vi "Get File Path.vi"(8 "error in (no error)":errorcluster caption="错误输入（无错误）", 10 "nRunMode":i32, 11 "nDevId":i32) -> (0 "error out":errorcluster caption="错误输出", 3 "function return":string)   [LabVIEW 2017, in "smncsftmt.lvlib"]
doc: "__declspec(dllexport) char* GetFilePath(int nDevId, int nRunMode);"
uses:
  smncsftmt.lvlib
  smncsftmt.dll
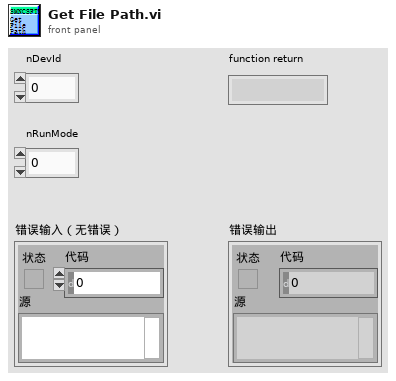
[diagram p1: front panel]
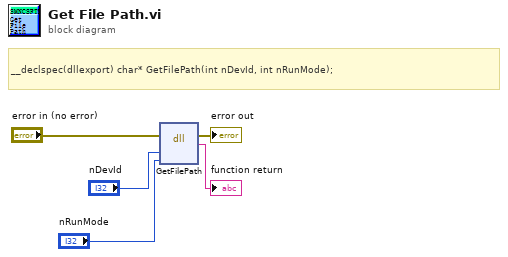
[diagram p0: block diagram]
diagram:
  # "__declspec(dllexport) char* GetFilePath(int nDevId, int nRunMode);"
  n1 = dll-call lib="PTH2oabs CUsersaDesktop\nLABVIEW范例National InstrumentsLabVIEW 2017user.lib\tsmncsftmtsmncsftmt.*" fn="GetFilePath"(error in="error in (no error)", "nDevId"="nDevId", "nRunMode"="nRunMode") -> (error out=→"error out":errorcluster, →"function return":string)  [unwired: 4 in, 1 out]
